vi "properties.get.vi"(8 "error in (no error)":errorcluster, 11 "asset in":refnum<class "asset.lvclass">) -> (0 "error out":errorcluster, 2 "properties":map{string, string}(c390), 3 "asset out":refnum<class "asset.lvclass">)   [LabVIEW 2020, in "asset.lvclass"]
uses:
  asset.lvclass
  asset.lvclass/asset.ctl
  nominal types/properties/properties.lvclass
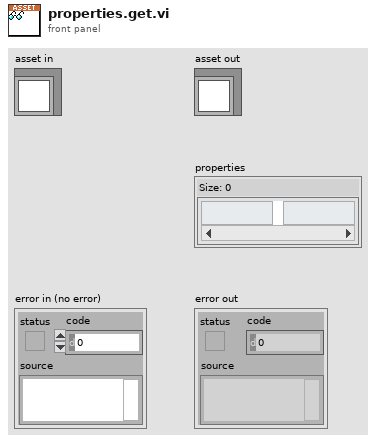
[diagram p1: front panel]
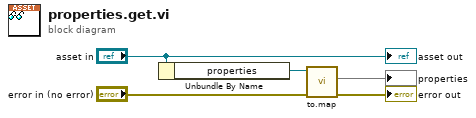
[diagram p0: block diagram]
diagram:
  n1 = Unbundle By Name("asset in") -> ("properties"=w1:refnum<class "properties.lvclass">)
  n2 = call "to.map.vi"("error in"="error in (no error)", "properties in"=w1) -> ("error out"=→"error out":errorcluster, "properties"=→"properties":map{string, string})  [unwired: 7 in, 1 out]
  "asset out" <- "asset in"
